vi "GetSetBinning.vi"(7 "Set?":bool, 8 "error in (no error)":errorcluster, 9 "dy in":i32, 10 "dx in":i32, 11 "Camera in":refnum<class "Camera.lvclass">) -> (0 "error out":errorcluster, 1 "dy out":i32, 2 "dx out":i32)   [LabVIEW 2020, in "Camera.lvclass"]
uses:
  Camera.lvclass
  Camera.lvclass/Camera.ctl
  bin/gindustrialcam_32-1.dll
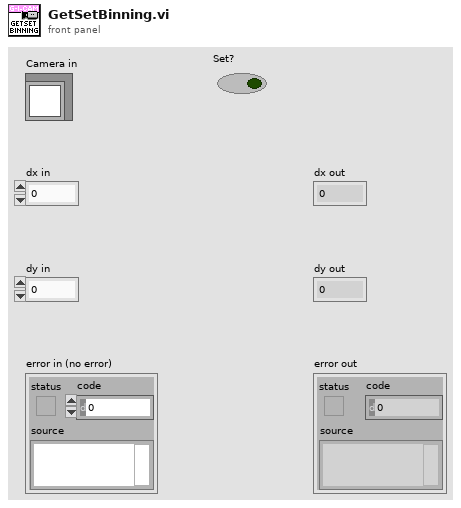
[diagram p1: front panel]
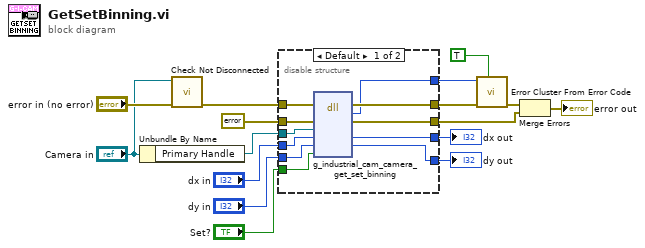
[diagram p0: block diagram]
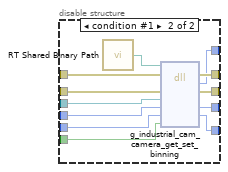
[diagram p2: hidden frame]
diagram:
  n1 = Unbundle By Name("Camera in") -> ("Primary Handle"=w7:refnum<data-value>)
  n2 = call "Check Not Disconnected.vi"("error in (no error)"="error in (no error)", "Camera in"="Camera in") -> ("error out"=w6:errorcluster)  [unwired: 9 in]
  n3 = disable-structure shown="Default" {
    disable-tunnel: [w27 w39] -> w16
    disable-tunnel: [w26 w38] -> w15
    disable-tunnel: [w25 w37] -> w13
    disable-tunnel: errorcluster {"status"=FALSE, "code"=0, "source"=""} ("error constant") -> [w24 w36]
    disable-tunnel: "Set?" -> [w23 w35]
    disable-tunnel: w7 -> [w22 w34]
    disable-tunnel: w6 -> [w21 w33]
    disable-tunnel: "dx in" -> [w20 w32]
    disable-tunnel: "dy in" -> [w19 w31]
    disable-tunnel: [w18 w30] -> w2
    disable-tunnel: [w17 w29] -> w1
    frame condition #0 (active) {
      n4 = dll-call lib="C:/serenial/lib/g-industrial-camera/LabVIEW/g_industrial_cam/bin/gindustrialcam_*-1.*" fn="g_industrial_cam_camera_get_set_binning"(error in=w21, "err"=w24, "edvr"=w22, "dx"=w20, "dy"=w19, "set"=w23) -> (error out=w27:errorcluster, "Mg_Error"=w26:i32, "err"=w25:errorcluster, "dx"=w18:i32, "dy"=w17:i32)  [unwired: 4 in, 1 out]
    }
    frame condition #1 {
      n5 = call "RT Shared Binary Path.vi"() -> ("Path"=w28:path)
      n6 = dll-call lib="C:/serenial/lib/g-industrial-camera/LabVIEW/g_industrial_cam/bin/gindustrialcam_*-1.*" fn="g_industrial_cam_camera_get_set_binning"(path in=w28, error in=w33, "err"=w36, "edvr"=w34, "dx"=w32, "dy"=w31, "set"=w35) -> (error out=w39:errorcluster, "Mg_Error"=w38:i32, "err"=w37:errorcluster, "dx"=w30:i32, "dy"=w29:i32)  [unwired: 3 in, 1 out]
    }
  }
  "dx out" <- w2
  "dy out" <- w1
  n7 = call <vilib>:"Error Cluster From Error Code.vi"("show call chain? (False)"=TRUE, "error in (no error)"=w16, "error code (0)"=w15) -> ("error out"=w14:errorcluster)  [unwired: 6 in]
  n8 = Merge Errors(w14, w13) -> (→"error out":errorcluster)
